vi "calculator.vi"(10 "y":dbl=3.0 caption="operand y", 11 "x":dbl=2.0 caption="operand x") -> (3 "x+y":dbl=5.0 caption="calculated result")   [LabVIEW 2021]
doc: "Deterministic numeric calculator VI for scientific automation via MCP. Use it for quick arithmetic checks, calibration offsets, parameter sanity checks, and reproducible test calculations before larger workflows. This version performs x plus y and returns the numeric result."
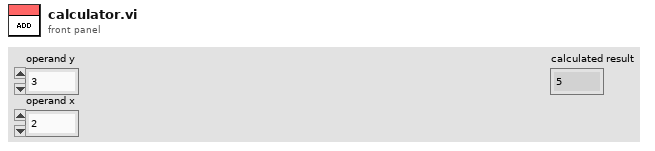
[diagram p1: front panel]
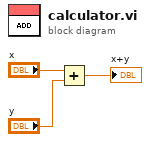
[diagram p0: block diagram]
diagram:
  n1 = Add(x="x", y="y") -> (x+y=→"x+y":dbl)
